vi "Handle Request.vi"(7 "Processing In":refnum<class "Processing.lvclass">, 11 "WebSocket Handler in":refnum<class "WebSocket Handler.lvclass">) -> (0 "error out":errorcluster, 5 "Processing":refnum<class "Processing.lvclass">)   [LabVIEW 2020, in "HTTP Server.lvlib" / "WebSocket Handler.lvclass"]
uses:
  WebSocket Handler.lvclass
  Processing/Processing.lvclass
  Processing/Processing.lvclass/Processing.ctl
  lv-http-util/HTTP Utils/Request/Request.lvclass/Request.ctl
  lv-uri/URI/URI/URI.lvclass/URI.ctl
  WebSocketUpgradeResponse/WebSocketUpgradeResponse.lvclass
  C:/dev/lv20CE/relink/lv-http-util/HTTP Utils/Response/Response.lvclass
  WebSocket Manager/WebSocket Manager.lvclass
  lv-http-util/HTTP Utils/Request/Request.lvclass
  lv-uri/URI/URI/URI.lvclass
  WebSocket Client/WebSocket Client.lvclass
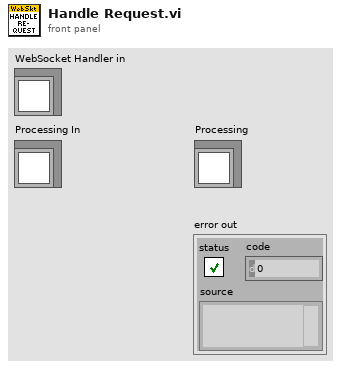
[diagram p1: front panel]
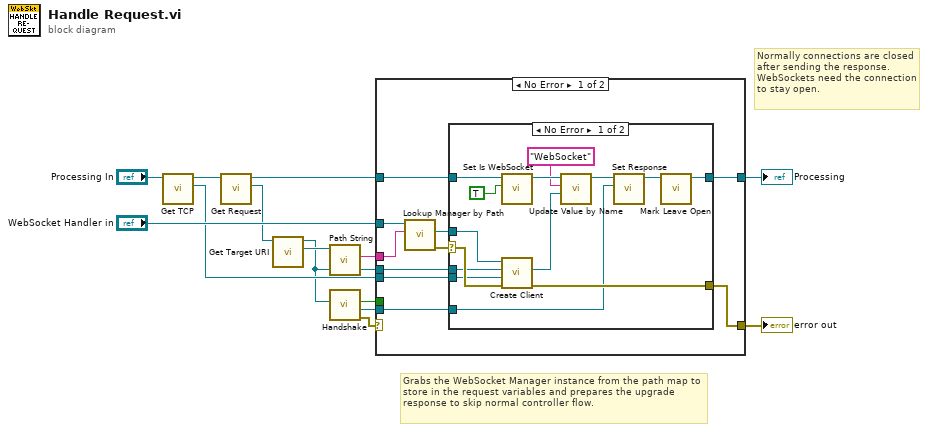
[diagram p0: block diagram]
diagram:
  # "Normally connections are closed after sending the response. WebSockets need the connection to stay open."
  # "Grabs the WebSocket Manager instance from the path map to store in the request variables and prepares the upgrade response to skip normal controller flow."
  n1 = call "Get TCP.vi"("Processing in"="Processing In") -> ("TCP"=w6:refnum<k5>, "Processing out"=w10:refnum<class "Processing.lvclass">)  [unwired: 9 in]
  n2 = call "Get Request.vi"("Processing in"=w10) -> ("Request"=w8:refnum<class "Request.lvclass">, "Processing out"=w12:refnum<class "Processing.lvclass">)  [unwired: 9 in]
  n3 = call "Get Target URI.vi"("Request in"=w8) -> ("Target URI"=w9:refnum<class "URI.lvclass">, "Request out"=w5:refnum<class "Request.lvclass">)  [unwired: 8 in, 1 out]
  n4 = call "Path String.vi"("URI in"=w9) -> ("Path String"=w7:string)  [unwired: 9 in, 1 out]
  n5 = call "Handshake.vi"("Request"=w5) -> ("error out"=w4:errorcluster, "Response out"=w1:refnum<class "WebSocketUpgradeResponse.lvclass">, "Is WS Upgrade"=w3:bool)  [unwired: 8 in]
  n6 = case shown="No Error" w4 {
    selector: w4 -> [_ w43]
    tunnel: [w23 w41] -> w14
    tunnel: w12 -> [w22 w41]
    tunnel: "WebSocket Handler in" -> [w21 _]
    tunnel: w7 -> [w20 _]
    tunnel: w6 -> [w18 _]
    tunnel: w5 -> [w17 _]
    tunnel: w3 -> [_ w44]
    tunnel: [w15 w42] -> w2
    tunnel: w1 -> [w16 _]
    frame No Error {
      n7 = call "Lookup Manager by Path.vi"("Path"=w20, "WebSocket Handler in"=w21) -> ("error out"=w24:errorcluster, "Manager"=w19:refnum<class "WebSocket Manager.lvclass">)  [unwired: 7 in, 1 out]
      n8 = case shown="No Error" w24 {
        selector: w24 -> [w37 w39]
        tunnel: [w36 w40] -> w23
        tunnel: w22 -> [w35 w40]
        tunnel: w19 -> [w34 _]
        tunnel: w18 -> [w33 _]
        tunnel: w17 -> [w27 _]
        tunnel: w16 -> [w26 _]
        tunnel: [w38 w39] -> w15
        frame No Error {
          n9 = call "Set Is WebSocket.vi"("Is WebSocket"=TRUE, "Processing in"=w35) -> ("Processing out"=w31:refnum<class "Processing.lvclass">)  [unwired: 9 in]
          n10 = call "Create Client.vi"("error in (no error)"=w37, "TCP"=w33, "Request"=w27, "WebSocket Manager in"=w34) -> ("error out"=w38:errorcluster, "WS Client"=w32:refnum<class "WebSocket Client.lvclass">)  [unwired: 6 in]
          n11 = call "Update Value by Name.vi"("Value"=w32, "Name"="WebSocket" ("Name / Service / Object"), "Processing in"=w31) -> ("Processing out"=w29:refnum<class "Processing.lvclass">)  [unwired: 7 in, 1 out]
          n12 = call "Set Response.vi"("Response"=w26, "Processing in"=w29) -> ("Processing out"=w30:refnum<class "Processing.lvclass">)  [unwired: 9 in]
          n13 = call "Mark Leave Open.vi"("Processing in"=w30) -> ("Processing out"=w36:refnum<class "Processing.lvclass">)  [unwired: 10 in]
        }
        frame Error {
        }
      }
    }
    frame Error {
      n14 = case shown="True" w44 {
        tunnel: w43 -> [_ w45]
        tunnel: [_ w45] -> w42
        frame False {
        }
        frame True {
        }
      }
    }
  }
  "error out" <- w2
  "Processing" <- w14
